vi "Launcher.vi"() -> ()   [LabVIEW 2025]
doc: "This is the top-level VI of this application. When it runs, it behaves like the splash screen many applications use to keep the user occupied while the application loads into memory. This application is quite small, so there is little overhead, which would make the splash screen just flash for a moment. Because that flash is distracting, there is a three-second delay inserted into this VI so that it stays up for a little bit. \n\nThis VI uses a delay-loaded subVI call to load the rest of the application. This trick ensures that the splash screen can load instantly regardless of how large the rest of the VI hierarchy gets, and the loading of the rest of the VIs becomes one step in the load process."
uses:
  ed69dc57-7765-441f-9a3c-b0af67f58143.vi
  Configuration Tools/Config Tool.lvlib
  Configuration Tools/SubVI/Load App.vi
panel:
  out "Engine Status":i32(listbox)=-1
  out "Title":string
  out "String":string
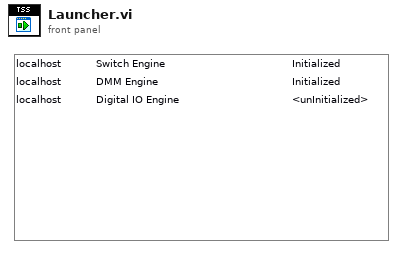
[diagram p1: front panel]
types:
  T1 = enum32{"Invalid", "Default", "Floating", "Floating/Auto-Hide", "Modal"}
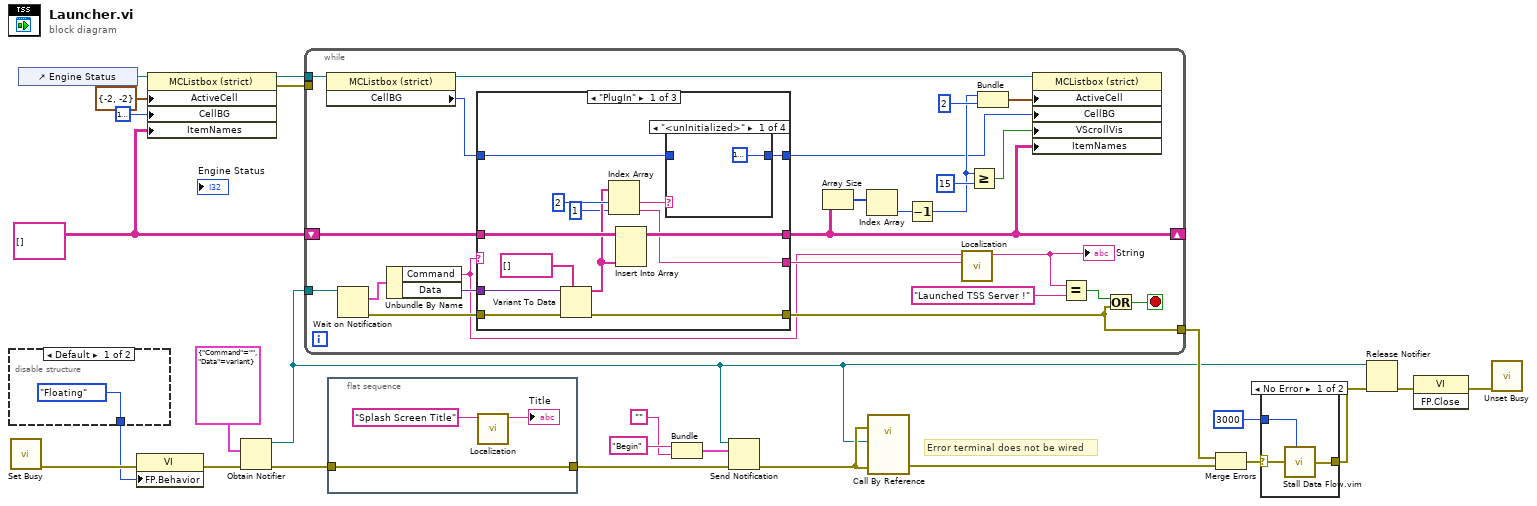
[diagram p0: block diagram]
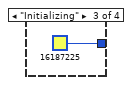
[diagram p3: hidden frame]
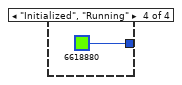
[diagram p4: hidden frame]
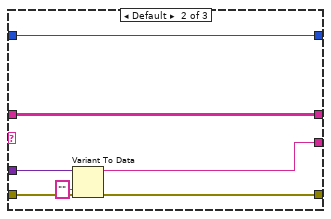
[diagram p5: hidden frame]
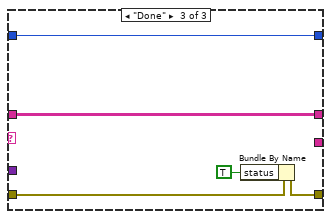
[diagram p6: hidden frame]
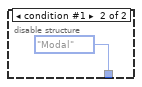
[diagram p7: hidden frame]
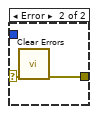
[diagram p8: hidden frame]
diagram:
  w9 = string[][] [] ("ItemNames")
  # "Error terminal does not be wired"
  n1 = disable-structure shown="Default" {
    disable-tunnel: [T1."Floating" ("Front Panel Window:Behavior") T1."Modal" ("Front Panel Window:Behavior")] -> w10
    frame condition #0 (active) {
    }
    frame condition #1 {
    }
  }
  n2 = call <vilib>:"Set Busy.vi"() -> ("error out"=w12:errorcluster)  [unwired: 10 in, 1 out]
  n3 = control-ref of="Engine Status"() -> (w16:refnum<vi>)
  n4 = property class="VI"(error in=w12, "FP.Behavior"=w10) -> (error out=w11:errorcluster)  [unwired: 1 in, 1 out]
  n5 = property class="MCListbox (strict)"(reference=w16, "ActiveCell"=cluster{"Row":i32, "Column":i32} {"Row"=-2, "Column"=-2} ("Active Cell:Active Cell"), "CellBG"=u32 16777216, "ItemNames"=w9) -> (reference out=w15:refnum<vi>, error out=w7:errorcluster)  [unwired: 1 in]
  n6 = Obtain Notifier(notification data type=cluster{"Command":string, "Data":variant} {"Command"="", "Data"=variant} ("Message Data"), error in (no error)=w11) -> (notifier out=w8:refnum<notifier>, error out=w3:errorcluster)  [unwired: 2 in, 1 out]
  n7 = while {
    tunnel: w8 -> [w50]
    tunnel: [w28] -> w22
    shift-right: [w36] -> _
    shift-left: w9 -> [w43]
    tunnel: w15 -> [w44]
    tunnel: w7 -> [_]
    stop <- w47 stop-if-true
    n8 = property class="MCListbox (strict)"(reference=w44) -> (reference out=w33:refnum<vi>, "CellBG"=w32:u32)  [unwired: 1 in, 1 out]
    n9 = Wait on Notification(notifier=w50) -> (notification=w45:cluster{"Command":string, "Data":variant}, error out=w29:errorcluster)  [unwired: 3 in, 2 out]
    n10 = Unbundle By Name(w45) -> ("Command"=w27:string, "Data"=w31:variant)
    n11 = case shown="\"PlugIn\"" w27 {
      tunnel: w31 -> [w56 w72 _]
      tunnel: w43 -> [w63 w74 w78]
      tunnel: [w59 w74 w78] -> w36
      tunnel: [w60 w73 w79] -> w34
      tunnel: w32 -> [w58 w73 w79]
      tunnel: [w51 w70 _] -> w30
      tunnel: w29 -> [w54 w69 w77]
      tunnel: [w53 w68 w75] -> w28
      frame "PlugIn" {
        n12 = Variant To Data(error in=w54, type=string[] [] ("ItemNames"), Variant=w56) -> (data=w55:string[], error out=w53:errorcluster)
        n13 = Index Array(array=w55, index #1=2 ("index"), index #2=1 ("index")) -> (element #1=w61:string, element #2=w51:string)
        n14 = Insert Into Array(array=w63, new element=w55) -> (w59:string[][])  [unwired: 2 in]
        n15 = case shown="\"<unInitialized>\"" w61 {
          tunnel: [u32 16777216 w65 u32 16187225 u32 6618880] -> w60
          tunnel: w58 -> [_ w65 _ _]
          frame "<unInitialized>" {
          }
          frame Default {
          }
          frame "Initializing" {
          }
          frame "Initialized", "Running" {
          }
        }
      }
      frame Default {
        n16 = Variant To Data(error in=w69, type="" ("Type"), Variant=w72) -> (data=w70:string, error out=w68:errorcluster)
      }
      frame "Done" {
        n17 = Bundle By Name(cluster=w77, "status"=TRUE) -> (w75:errorcluster)
      }
    }
    n18 = Array Size(array=w36) -> (size(s)=w39:i32[])
    n19 = Index Array(array=w39) -> (element=w40:i32)  [unwired: 1 in]
    n20 = Decrement(x=w40) -> (x-1=w37:i32)
    n21 = call "Localization.vi"("parameter"=w30, "Unlocalized"=w27) -> ("Localized"=w46:string)  [unwired: 9 in]
    "String" <- w46
    n22 = Greater Or Equal?(x=w37, y=15) -> (x >= y?=w35:bool)
    n23 = Bundle(w37, "disabled index (col)"=2) -> (w42:cluster{i32, "disabled index (col)":i32})  [unwired: 1 in]
    n24 = property class="MCListbox (strict)"(reference=w33, "ActiveCell"=w42, "CellBG"=w34, "VScrollVis"=w35, "ItemNames"=w36) -> ()  [unwired: 1 in, 2 out]
    n25 = Equal?(x=w46, y="Launched TSS Server !" ("notification")) -> (x = y?=w48:bool)
    n26 = Or(x=w48, y=w28) -> (x .or. y?=w47:bool)
  }
  n27 = flat-sequence {
    tunnel: w3 -> [w80]
    tunnel: [w80] -> w2
    frame #0 {
      n28 = call "Localization.vi"("Unlocalized"="Splash Screen Title" ("Window Title")) -> ("Localized"=→"Title":string)  [unwired: 10 in]
    }
  }
  n29 = Bundle("notification"="Begin", "") -> (w17:cluster{"notification":string, string})  [unwired: 1 in]
  n30 = Send Notification(notification=w17, notifier=w8, error in (no error)=w2) -> (error out=w21:errorcluster)  [unwired: 1 out]
  n31 = call-by-ref "?"(error in=w21, 8:"error in (no error)"=w21, "notifier"=w8) -> ("error out"=w20:errorcluster)  [unwired: 10 in, 2 out]
  n32 = Merge Errors(w22, w20) -> (w4:errorcluster)
  n33 = case shown="No Error" w4 {
    selector: w4 -> [w85 w86]
    tunnel: [w84 w87] -> w5
    tunnel: u32 3000 ("milliseconds to wait") -> [w83 _]
    frame No Error {
      n34 = call "Stall Data Flow.vim"("value in"=w85, "milliseconds to wait"=w83) -> ("value out"=w84:errorcluster)  [unwired: 1 out]
    }
    frame Error {
      n35 = call <vilib>:"Clear Errors.vi"("error in (no error)"=w86) -> ("error out"=w87:errorcluster)  [unwired: 5 in, 1 out]
    }
  }
  n36 = Release Notifier(notifier=w8, error in (no error)=w5) -> (error out=w24:errorcluster)  [unwired: 1 in, 2 out]
  n37 = invoke class="VI" method="FP.Close"(error in=w24) -> (error out=w23:errorcluster)  [unwired: 2 in, 2 out]
  n38 = call <vilib>:"Unset Busy.vi"("error in (no error)"=w23) -> ()  [unwired: 10 in, 1 out]
